vi "Afficher_profil.vi"(4 "Configuration":cluster{"Command (PV)":string, dbl}[](array[cluster]) {"?" format="%#.1f"}, 5 "Temps (s)":dbl[](array[numeric]) format="%#.1f", 6 "Températures (°C)":dbl[](array[numeric]) format="%#.1f", 7 "Evennements_entrée":T2) -> (0 "Graphe XY":cluster{"Y":dbl[], "Y":dbl[]}[](graph), 1 "Type de fin":string, 2 "Bornes profil":T1 {"Tempé. max" format="%#.1f"; "Tempé. min" format="%#.1f"; "Temps max" format="%#.1f"; "Temps min" format="%#.1f"}, 3 "Courbes à afficher":bool[](array[boolean]))   [LabVIEW 2022 SP3]
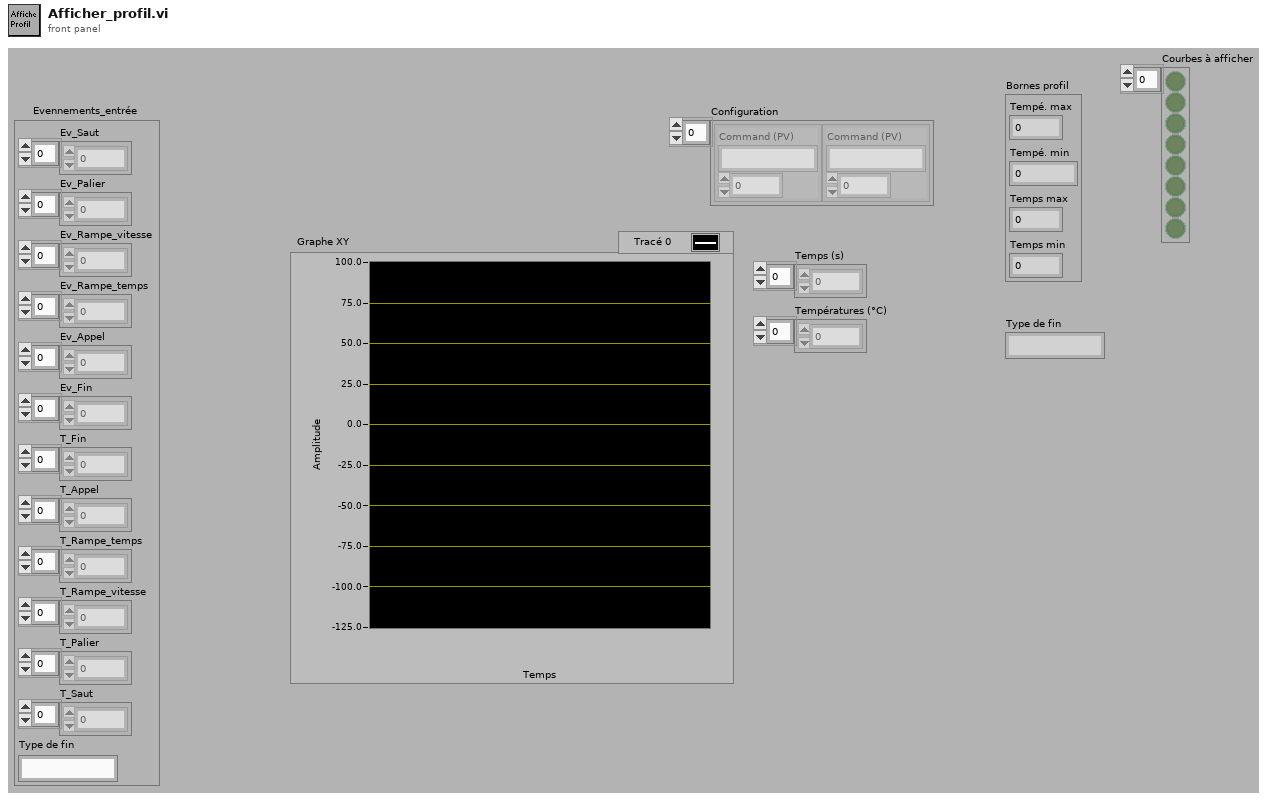
[diagram p1: front panel]
types:
  T1 = cluster{"Tempé. max":dbl, "Tempé. min":dbl, "Temps max":dbl, "Temps min":dbl}
  T2 = cluster{"Ev_Saut":dbl[], "Ev_Palier":dbl[], "Ev_Rampe_vitesse":dbl[], "Ev_Rampe_temps":dbl[], "Ev_Appel":dbl[], "Ev_Fin":dbl[], "T_Fin":dbl[], "T_Appel":dbl[], "T_Rampe_temps":dbl[], "T_Rampe_vitesse":dbl[], "T_Palier":dbl[], "T_Saut":dbl[], "Type de fin":string}
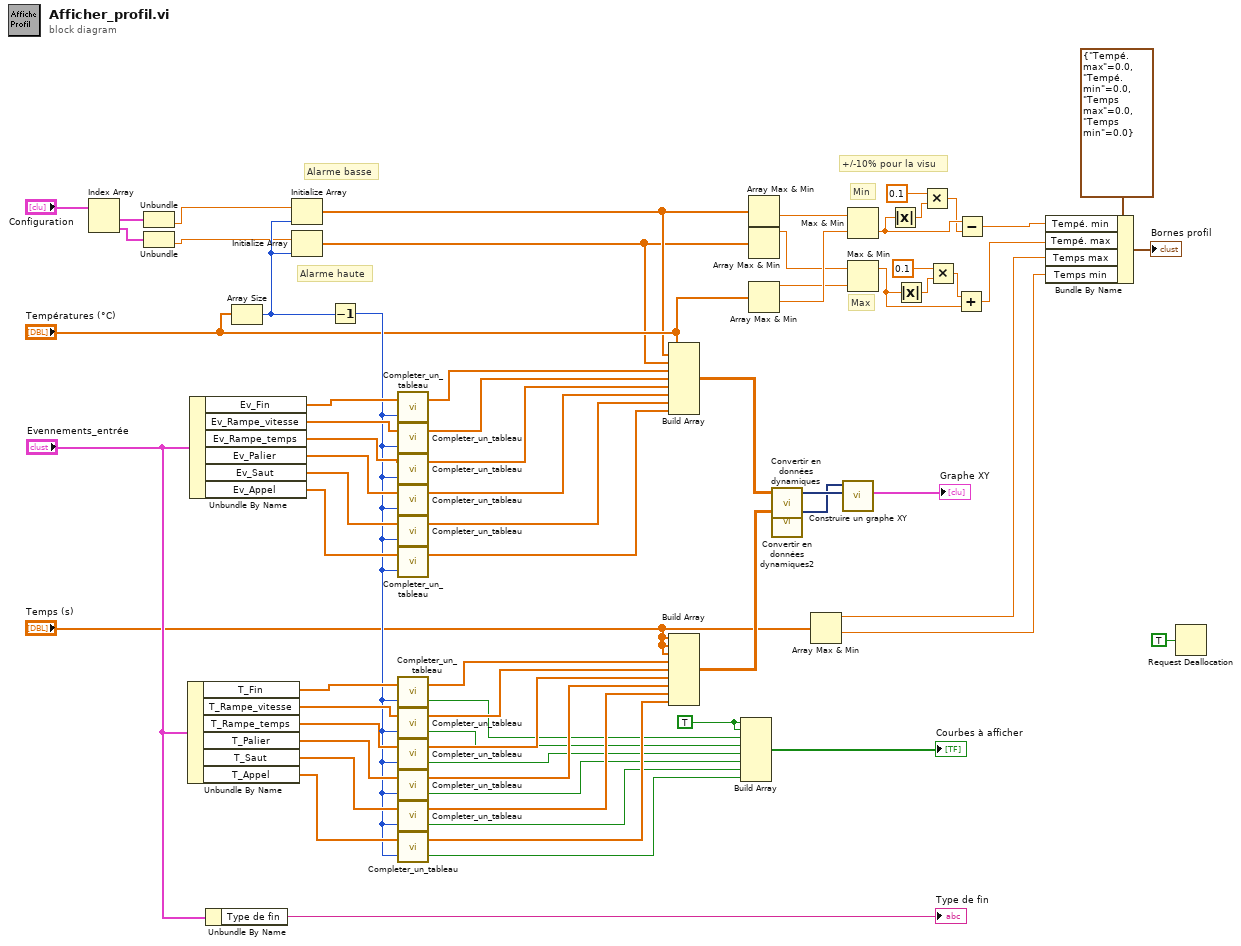
[diagram p0: block diagram]
diagram:
  w25 = TRUE
  # "+/-10% pour la visu"
  # "Max"
  # "Min"
  # "Alarme haute"
  # "Alarme basse"
  n1 = Index Array(array="Configuration") -> (element #1=w50:cluster{"Command (PV)":string, dbl}, element #2=w49:cluster{"Command (PV)":string, dbl})  [unwired: 2 in]
  n2 = Unbundle(w50) -> (w48:dbl)  [unwired: 1 out]
  n3 = Unbundle(w49) -> (w47:dbl)  [unwired: 1 out]
  n4 = Unbundle By Name("Evennements_entrée") -> ("T_Fin"=w64:dbl[], "T_Rampe_vitesse"=w63:dbl[], "T_Rampe_temps"=w62:dbl[], "T_Palier"=w61:dbl[], "T_Saut"=w60:dbl[], "T_Appel"=w59:dbl[])
  n5 = Unbundle By Name("Evennements_entrée") -> ("Ev_Fin"=w34:dbl[], "Ev_Rampe_vitesse"=w35:dbl[], "Ev_Rampe_temps"=w33:dbl[], "Ev_Palier"=w36:dbl[], "Ev_Saut"=w37:dbl[], "Ev_Appel"=w38:dbl[])
  n6 = Unbundle By Name("Evennements_entrée") -> ("Type de fin"=→"Type de fin":string)
  n7 = Array Size(array="Températures (°C)") -> (size(s)=w51:i32)
  n8 = Initialize Array(w48, w51) -> (w20:dbl[])
  n9 = Initialize Array(w47, w51) -> (w19:dbl[])
  n10 = Decrement(x=w51) -> (x-1=w24:i32)
  n11 = call "Completer_un_tableau.vi"("Remplir jusqu'à"=w24, "Tableau en entrée"=w34) -> ("Tableau en sortie"=w44:dbl[])  [unwired: 1 out]
  n12 = call "Completer_un_tableau.vi"("Remplir jusqu'à"=w24, "Tableau en entrée"=w35) -> ("Tableau en sortie"=w43:dbl[])  [unwired: 1 out]
  n13 = call "Completer_un_tableau.vi"("Remplir jusqu'à"=w24, "Tableau en entrée"=w33) -> ("Tableau en sortie"=w42:dbl[])  [unwired: 1 out]
  n14 = call "Completer_un_tableau.vi"("Remplir jusqu'à"=w24, "Tableau en entrée"=w36) -> ("Tableau en sortie"=w41:dbl[])  [unwired: 1 out]
  n15 = call "Completer_un_tableau.vi"("Remplir jusqu'à"=w24, "Tableau en entrée"=w37) -> ("Tableau en sortie"=w40:dbl[])  [unwired: 1 out]
  n16 = call "Completer_un_tableau.vi"("Remplir jusqu'à"=w24, "Tableau en entrée"=w38) -> ("Tableau en sortie"=w39:dbl[])  [unwired: 1 out]
  n17 = call "Completer_un_tableau.vi"("Remplir jusqu'à"=w24, "Tableau en entrée"=w64) -> ("Afficher ?"=w32:bool, "Tableau en sortie"=w58:dbl[])
  n18 = call "Completer_un_tableau.vi"("Remplir jusqu'à"=w24, "Tableau en entrée"=w63) -> ("Afficher ?"=w31:bool, "Tableau en sortie"=w57:dbl[])
  n19 = call "Completer_un_tableau.vi"("Remplir jusqu'à"=w24, "Tableau en entrée"=w62) -> ("Afficher ?"=w30:bool, "Tableau en sortie"=w56:dbl[])
  n20 = call "Completer_un_tableau.vi"("Remplir jusqu'à"=w24, "Tableau en entrée"=w61) -> ("Afficher ?"=w29:bool, "Tableau en sortie"=w55:dbl[])
  n21 = call "Completer_un_tableau.vi"("Remplir jusqu'à"=w24, "Tableau en entrée"=w60) -> ("Afficher ?"=w28:bool, "Tableau en sortie"=w54:dbl[])
  n22 = call "Completer_un_tableau.vi"("Remplir jusqu'à"=w24, "Tableau en entrée"=w59) -> ("Afficher ?"=w27:bool, "Tableau en sortie"=w53:dbl[])
  n23 = Build Array("Températures (°C)", w20, w19, w44, w43, w42, w41, w40, w39) -> (w68:dbl[][])
  n24 = Build Array("Temps (s)", "Temps (s)", "Temps (s)", w58, w57, w56, w55, w54, w53) -> (w66:dbl[][])
  n25 = Build Array(w25, w25, w32, w31, w30, w29, w28, w27) -> (→"Courbes à afficher":bool[])
  n26 = Array Max & Min(array=w20) -> (min value=w18:dbl)  [unwired: 3 out]
  n27 = Array Max & Min(array=w19) -> (max value=w15:dbl)  [unwired: 3 out]
  n28 = Array Max & Min(array="Températures (°C)") -> (max value=w16:dbl, min value=w17:dbl)  [unwired: 2 out]
  n29 = call "Convertir en données dynamiques"("2D Array"=w68) -> ("Dynamic Data Type"=w67:dynamicdata)  [unwired: 3 in]
  n30 = call "Convertir en données dynamiques2"("2D Array"=w66) -> ("Dynamic Data Type"=w65:dynamicdata)  [unwired: 3 in]
  n31 = Array Max & Min(array="Temps (s)") -> (max value=w3:dbl, min value=w2:dbl)  [unwired: 2 out]
  n32 = call "Construire un graphe XY"("Y Input"=w67, "X Input"=w65) -> ("XY Graph"=→"Graphe XY":cluster{"Y":dbl[], "Y":dbl[]}[])  [unwired: 8 in, 1 out]
  n33 = Max & Min(x=w18, y=w17) -> (min(x,y)=w5:dbl)  [unwired: 1 out]
  n34 = Max & Min(x=w15, y=w16) -> (max(x,y)=w7:dbl)  [unwired: 1 out]
  n35 = Absolute Value(x=w5) -> (abs(x)=w12:dbl)
  n36 = Absolute Value(x=w7) -> (abs(x)=w9:dbl)
  n37 = Multiply(x=0.1, y=w12) -> (x*y=w4:dbl)
  n38 = Multiply(x=0.1, y=w9) -> (x*y=w10:dbl)
  n39 = Add(x=w10, y=w7) -> (x+y=w6:dbl)
  n40 = Subtract(x=w5, y=w4) -> (x-y=w11:dbl)
  n41 = Bundle By Name(cluster=T1 {"Tempé. max"=0.0, "Tempé. min"=0.0, "Temps max"=0.0, "Temps min"=0.0} ("cluster d'entrée"), "Tempé. min"=w11, "Tempé. max"=w6, "Temps max"=w3, "Temps min"=w2) -> (→"Bornes profil":T1)
  n42 = Request Deallocation(TRUE ("flag")) -> ()
